vi "add module to engine.vi"(8 "error in":errorcluster, 10 "module ID":string, 11 "engine configuration in":refnum<class "engine configuration.lvclass">) -> (0 "error out":errorcluster, 3 "engine configuration out":refnum<class "engine configuration.lvclass">)   [LabVIEW 2014, in "engine configuration.lvclass"]
doc: "This function registers a module with the engine."
uses:
  engine configuration.lvclass
  engine configuration.lvclass/engine configuration.ctl
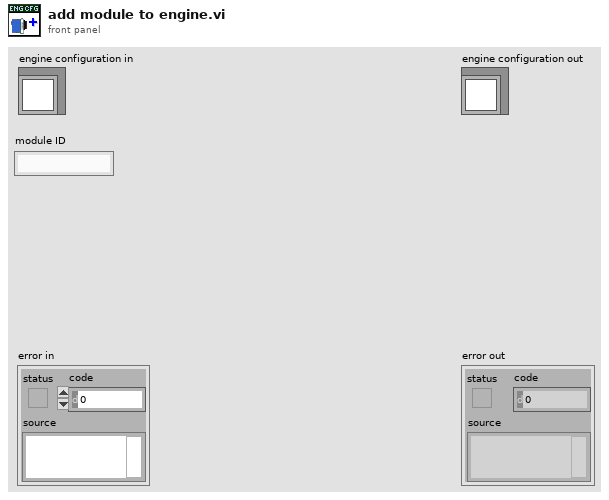
[diagram p1: front panel]
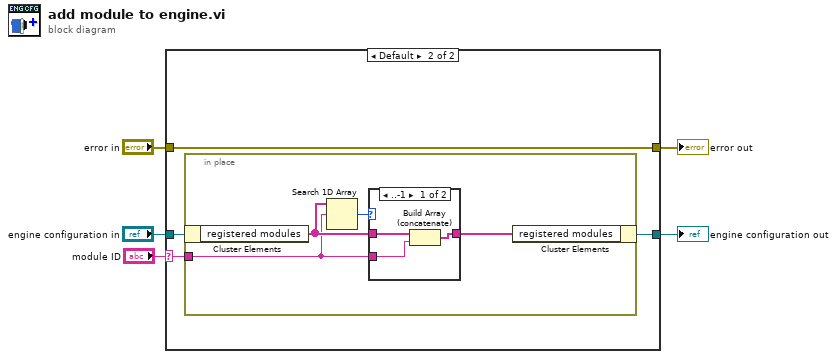
[diagram p0: block diagram]
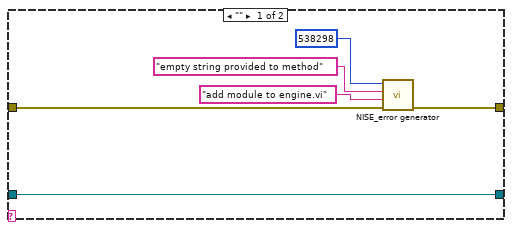
[diagram p2: hidden frame]
diagram:
  n1 = case shown="Default" "module ID" {
    selector: "module ID" -> [_ w13]
    tunnel: "engine configuration in" -> [w11 w15]
    tunnel: [w11 w14] -> w4
    tunnel: [w9 w12] -> w2
    tunnel: "error in" -> [w8 w12]
    frame "" {
      n2 = call <vilib>:"NISE_error generator.vi"("error in"=w8, "source"="add module to engine.vi", "append error message"="empty string provided to method", "error code (0)"=538298) -> ("error out"=w9:errorcluster)  [unwired: 5 in]
    }
    frame Default {
      n3 = in-place {
        in-place-border: w13 -> [w16]
        n4 = in-place-cluster #1(w15) -> ("registered modules"=w17:string[])
        n5 = Search 1D Array(1D array=w17, element=w16) -> (index of element=w19:i32)  [unwired: 1 in]
        n6 = case shown="..-1" w19 {
          tunnel: [w22 w23] -> w18
          tunnel: w17 -> [w21 w23]
          tunnel: w16 -> [w20 _]
          frame ..-1 {
            n7 = Build Array (concatenate)(w21, w20) -> (w22:string[])
          }
          frame 0.. {
          }
        }
        n8 = in-place-cluster #1("registered modules"=w18) -> (w14:refnum<class "engine configuration.lvclass">)
      }
    }
  }
  "engine configuration out" <- w4
  "error out" <- w2
